vi "xlsx to Cluster (Ballard - 1553).vi"(8 "Error (in)":errorcluster, 11 "file path (dialog if empty)":path) -> (0 "Error (out)":errorcluster, 2 "Configuration Array":T3[](array[typedef]), 3 "hw configuration":T1[](array[typedef]))   [LabVIEW 2020]
uses:
  _controls/ballard1553_cluster.ctl
  _controls/aim1553_messages.ctl
  _controls/1553_Parameters_key.ctl
  _controls/1553_Parameters.ctl
  _controls/1553_minorFrames.ctl
  _controls/ballard1553_hw_map.ctl
  _controls/ballard1553_RT_list.ctl
panel:
  out "data":string[][](array[string])
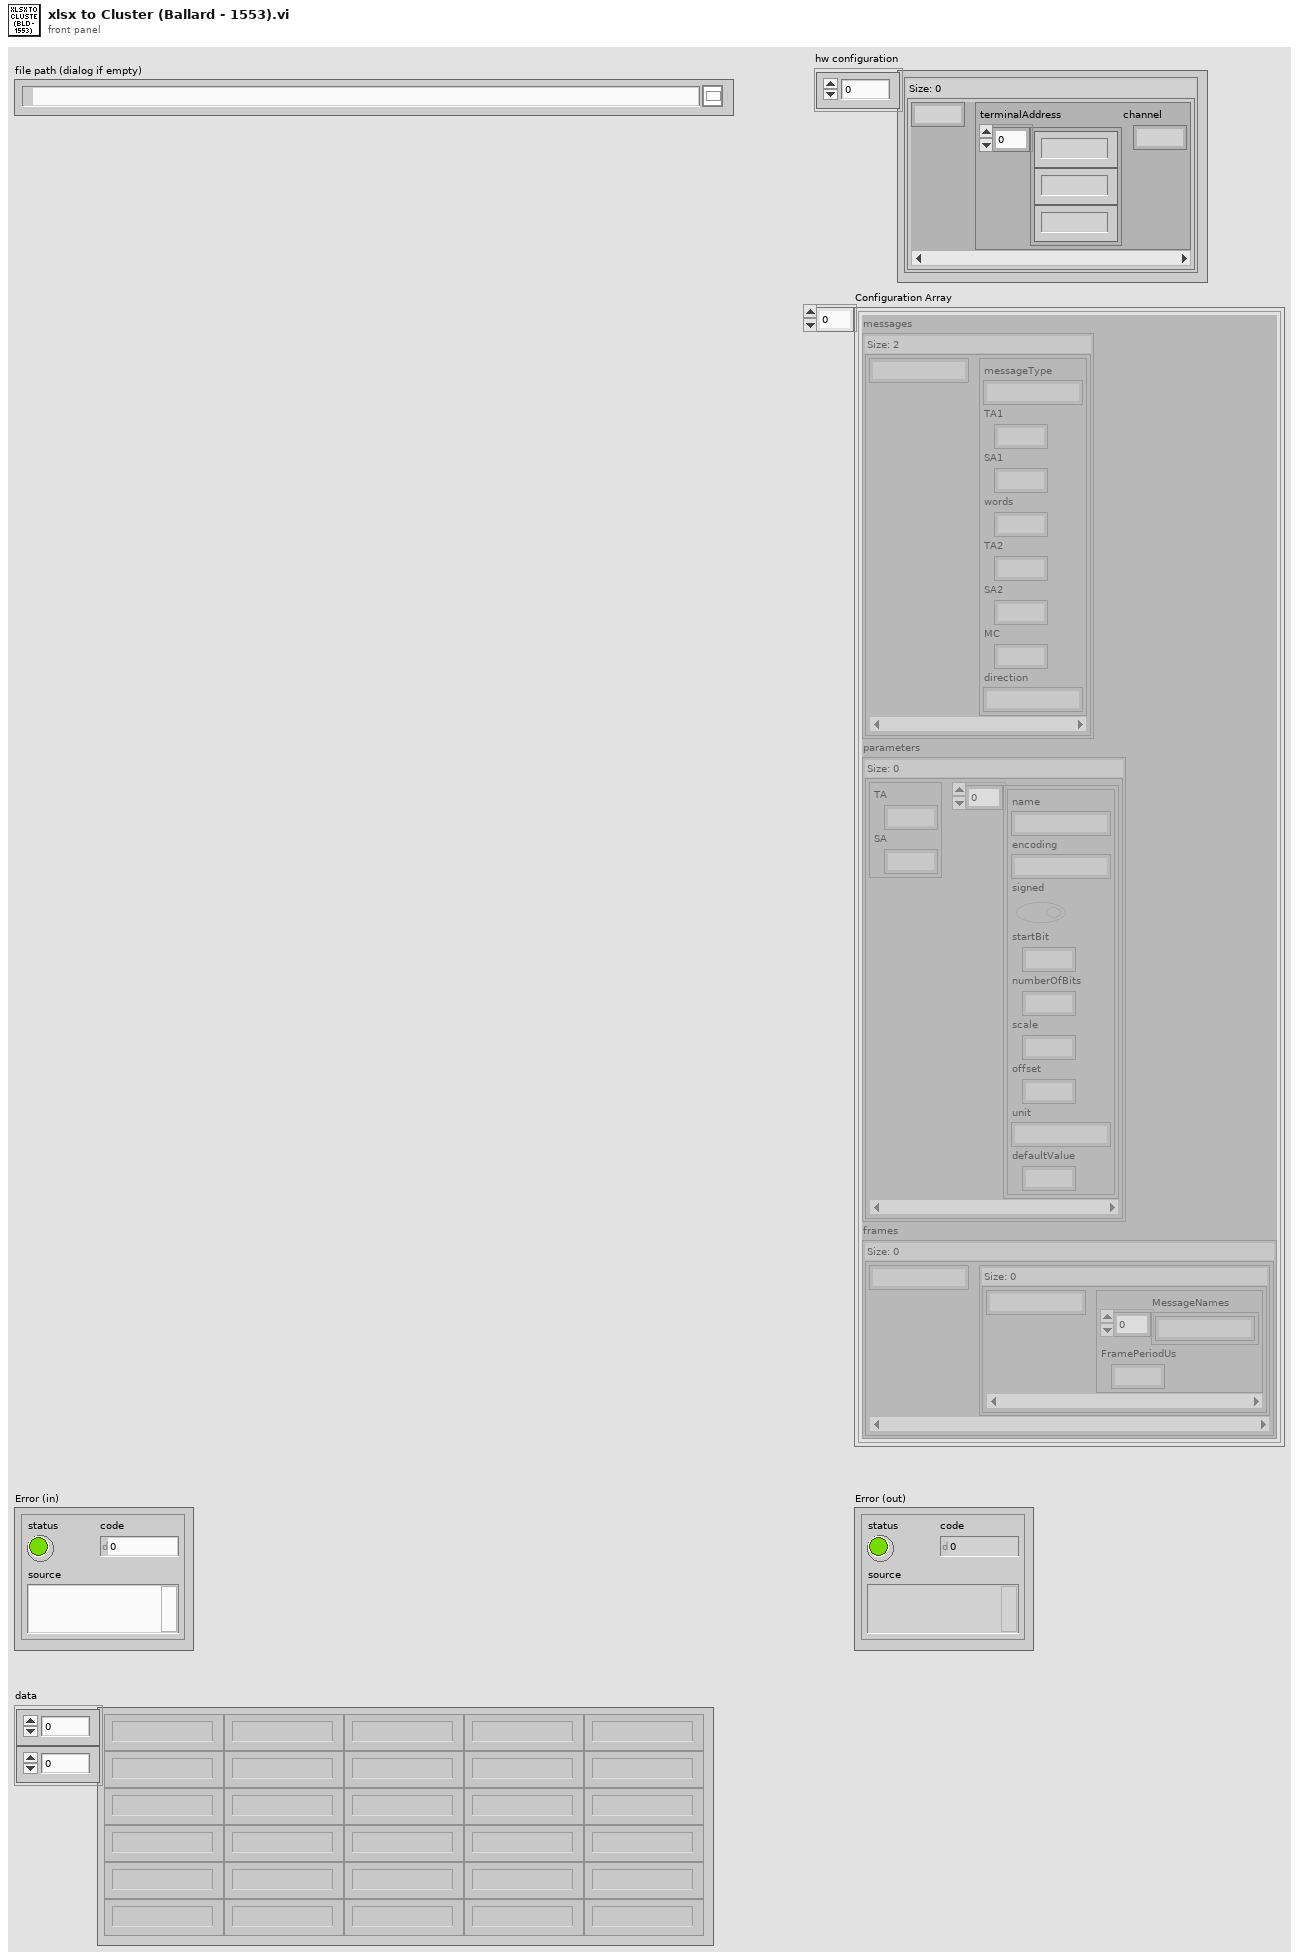
[diagram p1: front panel]
types:
  T1 = typedef "ballard1553_hw_map.ctl" = map{i32, T2}
  T2 = typedef "ballard1553_RT_list.ctl" = cluster{"terminalAddress":i32[], "channel":i32}
  T3 = typedef "ballard1553_cluster.ctl" = cluster{"messages":map{string, T4}, "parameters":map{T5, T6[]}, "frames":map{string, map{string, T7}}}
  T4 = typedef "aim1553_messages.ctl" = cluster{"messageType":string, "TA1":i32, "SA1":i32, "words":i32, "TA2":i32, "SA2":i32, "MC":i32, "direction":string}
  T5 = typedef "1553_Parameters_key.ctl" = cluster{"TA":i32, "SA":i32}
  T6 = typedef "1553_Parameters.ctl" = cluster{"name":string, "encoding":string, "signed":bool, "startBit":i32, "numberOfBits":i32, "scale":dbl, "offset":dbl, "unit":string, "defaultValue":dbl}
  T7 = typedef "1553_minorFrames.ctl" = cluster{"MessageNames":string[], "FramePeriodUs":i32}
  T8 = typedef "excelRefContainer.ctl" = cluster{"Application":refnum<k7>, "Workbooks":refnum<k7>, "Workbook":refnum<k7>}
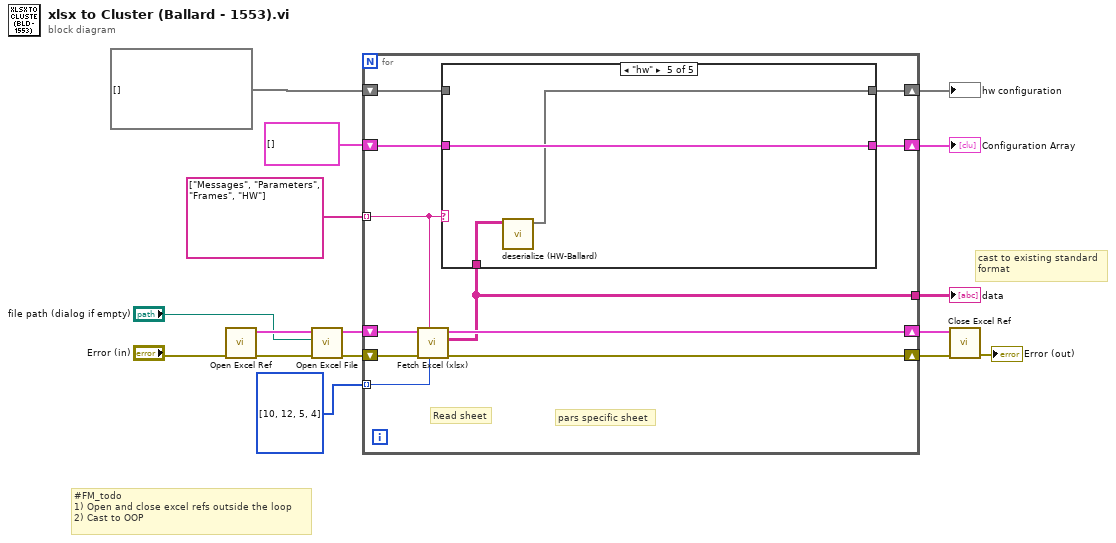
[diagram p0: block diagram]
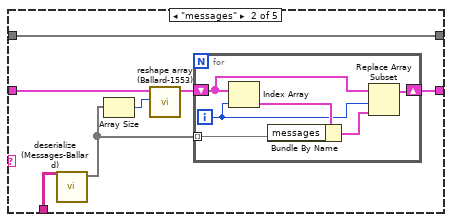
[diagram p3: hidden frame]
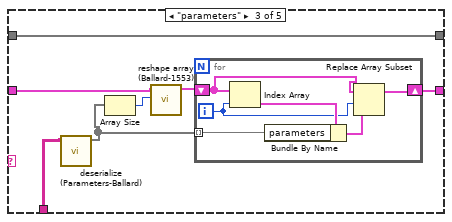
[diagram p4: hidden frame]
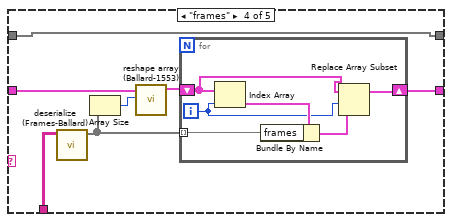
[diagram p5: hidden frame]
diagram:
  # "#FM_todo\n1) Open and close excel refs outside the loop\n2) Cast to OOP"
  # "cast to existing standard\nformat"
  n1 = call "Open Excel Ref.vi"("error in"="Error (in)") -> ("error out"=w12:errorcluster, "excelRefs out"=w11:T8)  [unwired: 9 in]
  n2 = call "Open Excel File.vi"("error in"=w12, "file path"="file path (dialog if empty)", "excelRefs in"=w11) -> ("error out"=w8:errorcluster, "excelRefs out"=w7:T8)  [unwired: 7 in]
  n3 = for {
    shift-right: [w25] -> w13
    shift-left: w8 -> [w24]
    tunnel: string[] ["Messages", "Parameters", "Frames", "HW"] -> [w22] mode=indexing
    tunnel: [w21] -> w15
    tunnel: i32[] [10, 12, 5, 4] ("columns (21)") -> [w23] mode=indexing
    shift-right: [w26] -> w5
    shift-left: w7 -> [w27]
    shift-right: [w19] -> w4
    shift-left: T3[] [] -> [w20]
    shift-right: [w17] -> w1
    shift-left: T1[] [] ("hw configuration") -> [w18]
    # "pars specific sheet"
    # "Read sheet"
    n4 = call "Fetch Excel (xlsx).vi"("columns (21)"=w23, "Excel._SheetName"=w22, "error in (no error)"=w24, "excelRefs in"=w27) -> ("error out"=w25:errorcluster, "data"=w21:string[][], "excelRefs out"=w26:T8)  [unwired: 5 in]
    n5 = case shown="\"hw\"" w22 {
      tunnel: w21 -> [_ w31 w44 w57 w70]
      tunnel: w20 -> [w28 w33 w47 w61 w71]
      tunnel: [w28 w34 w46 w62 w71] -> w19
      tunnel: w18 -> [w29 w32 w45 w58 _]
      tunnel: [w29 w32 w45 w58 w69] -> w17
      frame Default {
      }
      frame "messages" {
        n6 = call "deserialize (Messages-Ballard).vi"("data in"=w31) -> ("messages"=w30:map{string, T4}[])  [unwired: 10 in]
        n7 = Array Size(array=w30) -> (size(s)=w35:i32)
        n8 = call "reshape array (Ballard-1553).vi"("size requested"=w35, "Array in"=w33) -> ("Array out"=w36:T3[])  [unwired: 9 in]
        n9 = for {
          shift-right: [w38] -> w34
          shift-left: w36 -> [w41]
          tunnel: w30 -> [w37] mode=indexing
          i -> [w40]
          n10 = Index Array(array=w41, index=w40) -> (element=w42:T3)
          n11 = Bundle By Name(cluster=w42, "messages"=w37) -> (w39:T3)
          n12 = Replace Array Subset(array=w41, new element=w39, index=w40) -> (w38:T3[])
        }
      }
      frame "parameters" {
        n13 = call "deserialize (Parameters-Ballard).vi"("data in"=w44) -> ("parameters out"=w43:map{T5, T6[]}[])  [unwired: 10 in]
        n14 = Array Size(array=w43) -> (size(s)=w48:i32)
        n15 = call "reshape array (Ballard-1553).vi"("size requested"=w48, "Array in"=w47) -> ("Array out"=w49:T3[])  [unwired: 9 in]
        n16 = for {
          shift-right: [w50] -> w46
          shift-left: w49 -> [w53]
          tunnel: w43 -> [w54] mode=indexing
          i -> [w52]
          n17 = Index Array(array=w53, index=w52) -> (element=w55:T3)
          n18 = Bundle By Name(cluster=w55, "parameters"=w54) -> (w51:T3)
          n19 = Replace Array Subset(array=w53, new element=w51, index=w52) -> (w50:T3[])
        }
      }
      frame "frames" {
        n20 = call "deserialize (Frames-Ballard).vi"("data in"=w57) -> ("frames"=w56:map{string, map{string, T7}}[])  [unwired: 10 in]
        n21 = Array Size(array=w56) -> (size(s)=w59:i32)
        n22 = call "reshape array (Ballard-1553).vi"("size requested"=w59, "Array in"=w61) -> ("Array out"=w60:T3[])  [unwired: 9 in]
        n23 = for {
          shift-right: [w63] -> w62
          shift-left: w60 -> [w66]
          tunnel: w56 -> [w67] mode=indexing
          i -> [w65]
          n24 = Index Array(array=w66, index=w65) -> (element=w68:T3)
          n25 = Bundle By Name(cluster=w68, "frames"=w67) -> (w64:T3)
          n26 = Replace Array Subset(array=w66, new element=w64, index=w65) -> (w63:T3[])
        }
      }
      frame "hw" {
        n27 = call "deserialize (HW-Ballard).vi"("data in"=w70) -> ("hw configuration"=w69:T1[])  [unwired: 10 in]
      }
    }
  }
  "data" <- w15
  "Configuration Array" <- w4
  "hw configuration" <- w1
  n28 = call "Close Excel Ref.vi"("error in"=w13, "excelRefs in"=w5) -> ("error out"=→"Error (out)":errorcluster)  [unwired: 9 in]
